vi "Assert Greater_Variant.vi"(4 "Execution time (s)":dbl=-1.0, 5 "Assert Only? (F)":bool, 6 "error code (1)":i32=1, 7 "Label":string, 8 "error in (no error)":errorcluster, 9 "Register with caller test (F)":bool, 10 "Y":variant, 11 "X":variant) -> (0 "error out":errorcluster, 2 "Properties.Assert":refnum<class "Properties.Assert.lvclass">)   [LabVIEW 2013, in "Caraya.lvlib" / "Assert.lvclass"]
doc: "Generates an error if the input condition is not met.\n\n--\nCopyright © 2015 JKI All rights reserved.\n\nAuthor: Tomi Maila <tomi.maila@jki.net>\n\nThis library is provided \"AS IS\" ,WITHOUT WARRANTIES OR\nCONDITIONS OF ANY KIND, either express or implied.\n\nJKI -- jki.net"
uses:
  Assert.lvclass
  Properties.Assert/Properties.Assert.lvclass
  Properties/Properties.lvclass
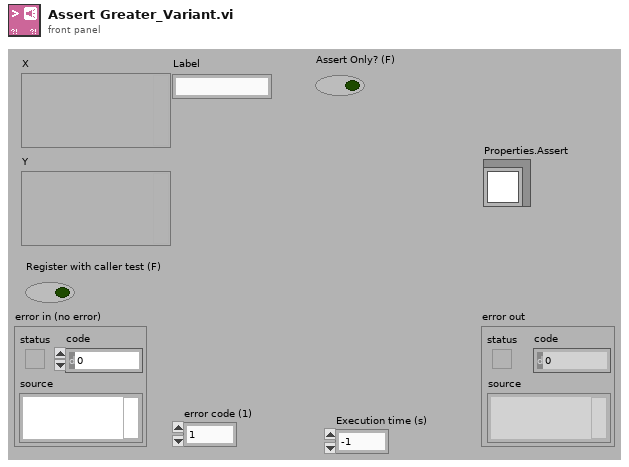
[diagram p1: front panel]
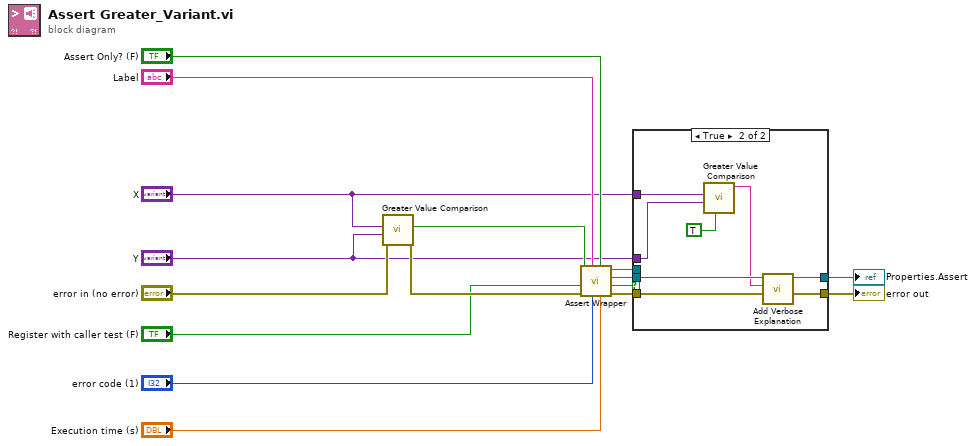
[diagram p0: block diagram]
diagram:
  n1 = call "Greater Value Comparison.vi"("error in (no error)"="error in (no error)", "Y"="Y", "X"="X") -> ("error out"=w8:errorcluster, "Asserted?"=w7:bool)  [unwired: 6 in, 1 out]
  n2 = call "Assert Wrapper.vi"("Execution time (s)"="Execution time (s)", "Assert Only? (F)"="Assert Only? (F)", "error code (1)"="error code (1)", "Label"="Label", "error in (no error)"=w8, "Register with caller test (F)"="Register with caller test (F)", "Assert?"=w7) -> ("error out"=w11:errorcluster, "Verbose"=w10:bool, "Properties.Assert"=w2:refnum<class "Properties.Assert.lvclass">, "Assert out"=w3:refnum<class "Assert.lvclass">)  [unwired: 1 in]
  n3 = case shown="True" w10 {
    tunnel: [w18 w21] -> w12
    tunnel: w3 -> [_ _]
    tunnel: w11 -> [w18 w22]
    tunnel: "X" -> [_ w25]
    tunnel: "Y" -> [_ w24]
    tunnel: w2 -> [w17 w23]
    tunnel: [w17 w19] -> w1
    frame False {
    }
    frame True {
      n4 = call "Greater Value Comparison.vi"("verbose? (F)"=TRUE, "Y"=w24, "X"=w25) -> ("Verbose output"=w20:string)  [unwired: 6 in, 2 out]
      n5 = call "Add Verbose Explanation.vi"("error in (no error)"=w22, "Verbose Explanation"=w20, "Properties"=w23) -> ("error out"=w21:errorcluster, "Properties"=w19:refnum<class "Properties.Assert.lvclass">)  [unwired: 7 in]
    }
  }
  "error out" <- w12
  "Properties.Assert" <- w1
